vi "ziTicks2S.vi"   [LabVIEW 2009, in "Zurich Instruments LabOne.lvlib"]
doc: "Convert a scalara or vector value from the machine unit ticks to the SI unit second."
uses:
  <instrlib>/Zurich Instruments LabOne/Zurich Instruments LabOne.lvlib
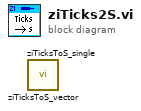
[diagram p0: block diagram]
diagram:
  n1 = call <instrlib>:"ziTicksToS_vector.vi"() -> ()  [unwired: 3 in, 3 out]
  n2 = call <instrlib>:"ziTicksToS_single.vi"() -> ()  [unwired: 3 in, 3 out]
